vi "Tree_ItemArrayTag_Tests.vi"(11 "error in":errorcluster) -> (15 "error out":errorcluster)   [LabVIEW 2016, in "DronaTest.lvlib"]
uses:
  DronaTest.lvlib
  APIs/Stimulus/ControlValue/SetValueAuto.vi
  APIs/Stimulus/ControlValue/Controls/Tree/SetValueByItemTagArray.vi
  APIs/Assert/AssertControlValue/Equal.vi
  <vilib>/addons/_JKI Toolkits/Caraya/classes/Test/Test.lvclass
  Drona.lvlib
  <vilib>/SLL Toolkit/SLL Debug/SLL Debug.lvlib
  APIs/Assert/AssertControlValue/AssertControlValue.lvlib
  APIs/Stimulus/ControlValue/ControlValue.lvlib
  <vilib>/addons/_JKI Toolkits/Caraya/classes/Assert/Assert.lvclass
  APIs/Stimulus/ControlValue/Controls/Tree/StimulusTree.lvlib
  APIs/Get/GetControlRef/GetControlRef.lvlib
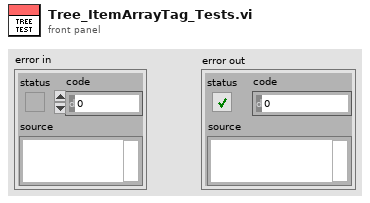
[diagram p1: front panel]
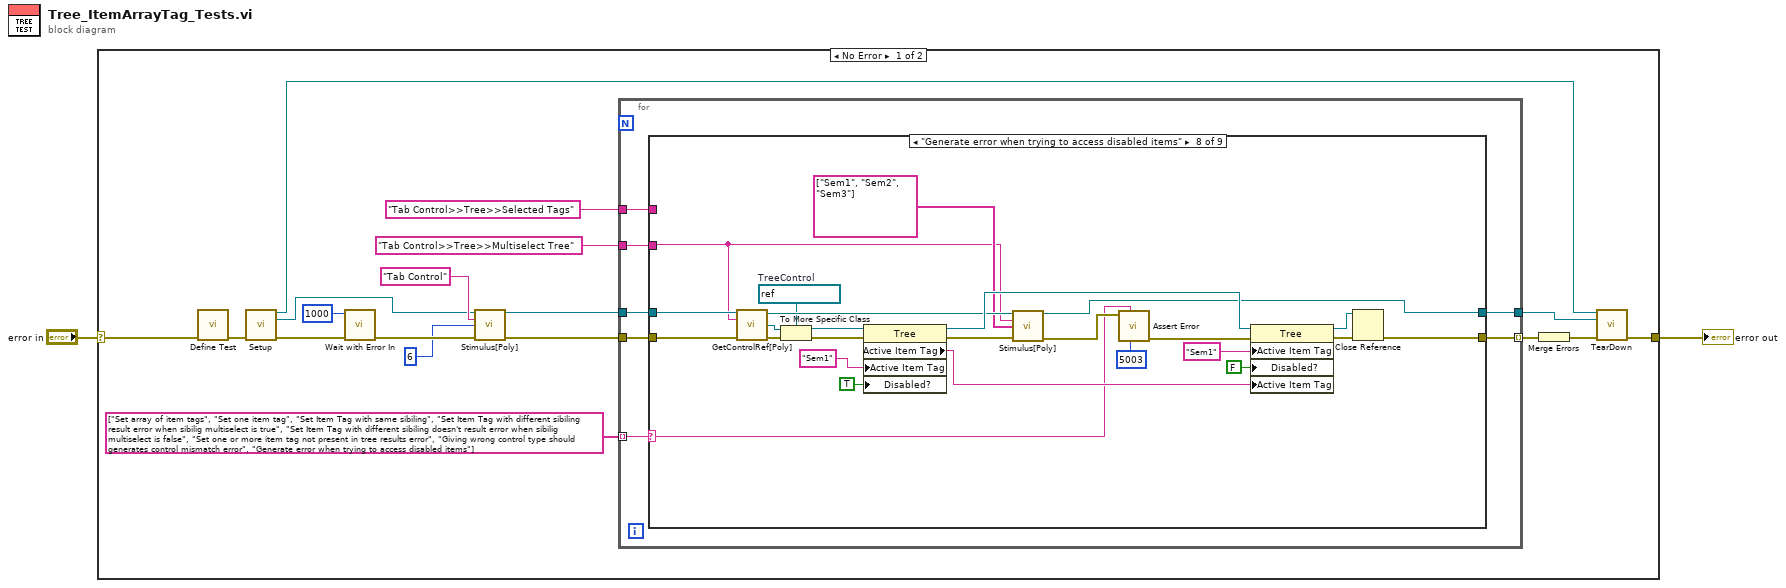
[diagram p0: block diagram]
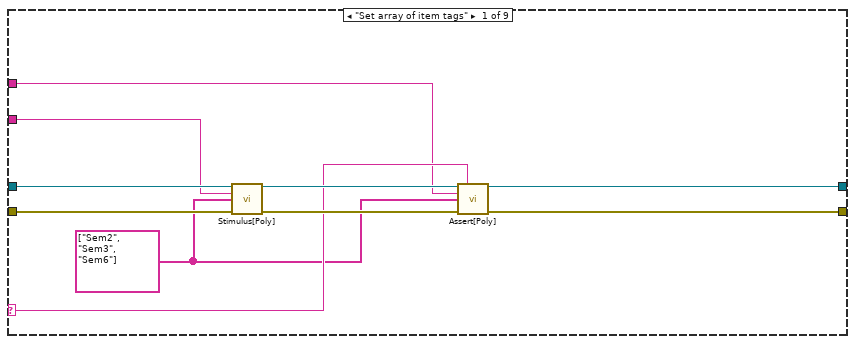
[diagram p2: hidden frame]
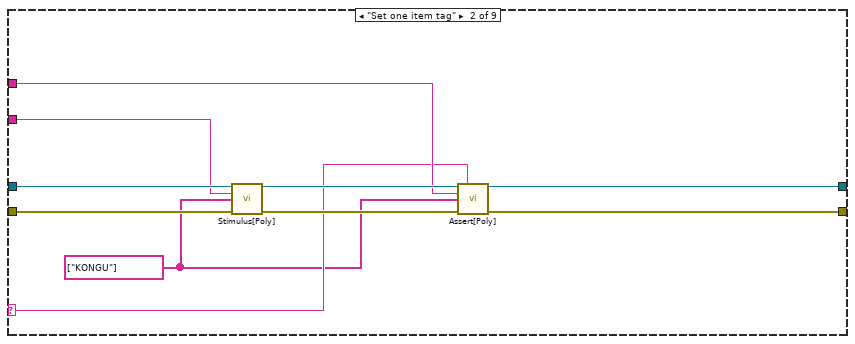
[diagram p3: hidden frame]
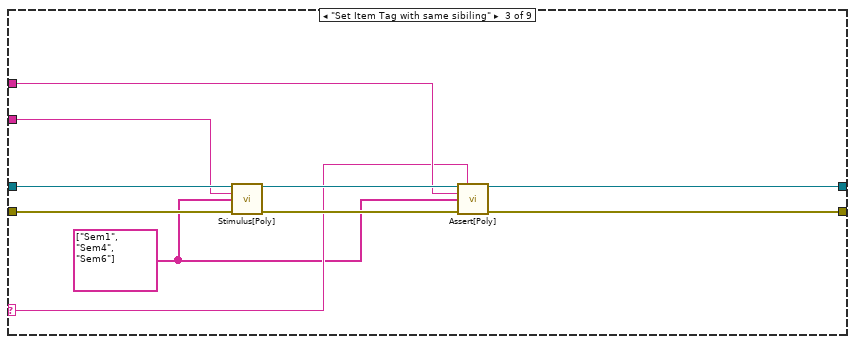
[diagram p4: hidden frame]
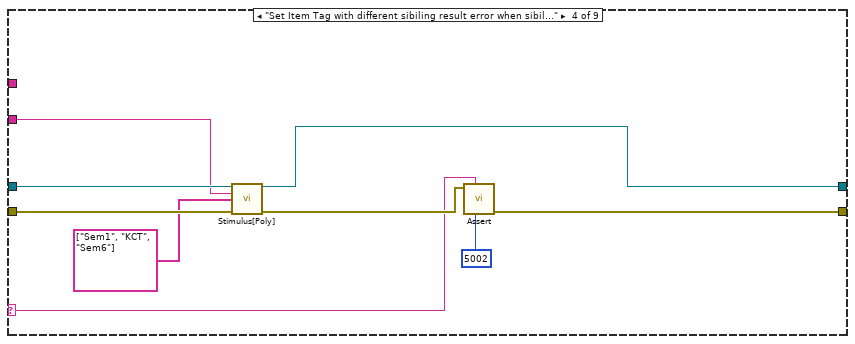
[diagram p5: hidden frame]
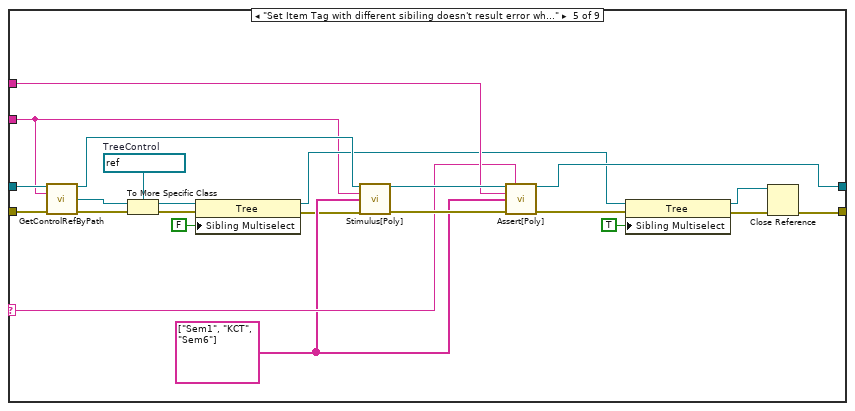
[diagram p6: hidden frame]
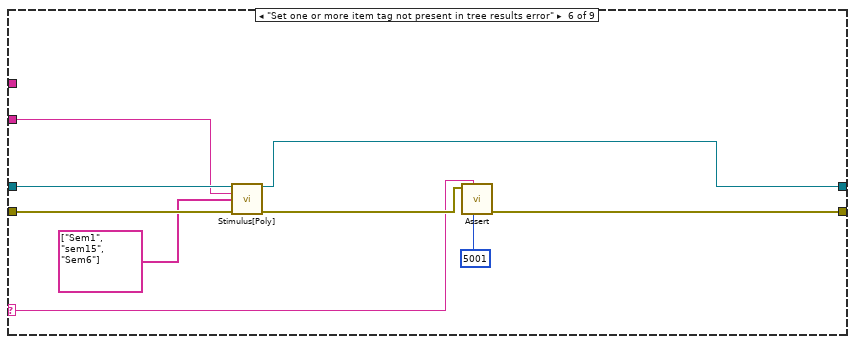
[diagram p7: hidden frame]
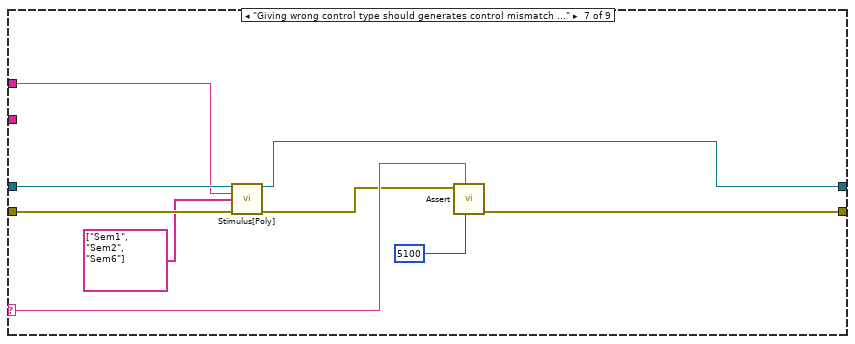
[diagram p8: hidden frame]
diagram:
  n1 = case shown="No Error" "error in" {
    selector: "error in" -> [w20 w135]
    tunnel: [w3 w135] -> w1
    frame No Error {
      n2 = call <vilib>:"Define Test.vi"("error in (no error)"=w20) -> ("error out"=w9:errorcluster)  [unwired: 9 in, 1 out]
      n3 = call "Setup.vi"("error in"=w9) -> ("Application Ref"=w4:refnum<vi>, "VI out"=w8:refnum<vi>, "error out"=w7:errorcluster)  [unwired: 12 in]
      n4 = call <vilib>:"Wait with Error In.vi"("error in (no error)"=w7, "milliseconds to wait"=u32 1000) -> ("error out"=w18:errorcluster)  [unwired: 9 in]
      n5 = call-poly "Stimulus[Poly].vi"("VI Reference In"=w8, "Control Path"="Tab Control", "Value (Signaling)"=6, "error in"=w18) -> ("VI Reference Out"=w14:refnum<vi>, "error out"=w17:errorcluster)  [unwired: 10 in]
      n6 = for {
        tunnel: w14 -> [w26]
        tunnel: "Tab Control>>Tree>>Multiselect Tree" ("Control Path") -> [w25]
        tunnel: "Tab Control>>Tree>>Selected Tags" ("Control Path") -> [w24]
        tunnel: string[] ["Set array of item tags", "Set one item tag", "Set Item Tag with same sibiling", "Set Item Tag with different sibiling result error when sibilig multiselect is true", "Set Item Tag with different sibiling doesn't result error when sibilig multiselect is false", "Set one or more item tag not present in tree results error", "Giving wrong control type should generates control mismatch error", "Generate error when trying to access disabled items"] -> [w22] mode=indexing
        tunnel: [w21] -> w5
        tunnel: w17 -> [w27]
        tunnel: [w23] -> w10 mode=indexing
        n7 = case shown="\"Generate error when trying to access disabled items\"" w22 {
          selector: w22 -> [w31 w39 w49 w61 w85 w92 w104 w110 _]
          tunnel: w27 -> [w37 w47 w57 w66 w83 w98 w107 w114 w134]
          tunnel: w26 -> [w36 w46 w56 w65 w82 w97 w106 w113 w133]
          tunnel: w25 -> [w29 w43 w53 w64 w67 w96 _ w108 _]
          tunnel: w24 -> [w30 w42 w52 _ w87 _ w100 _ _]
          tunnel: [w33 w41 w51 w59 w69 w95 w105 w112 w134] -> w23
          tunnel: [w32 w40 w50 w58 w86 w94 w103 w111 w133] -> w21
          frame "Set array of item tags" {
            w28 = string[] ["Sem2", "Sem3", "Sem6"] ("Item Name")
            n8 = call-poly "Stimulus[Poly].vi"("VI Reference In"=w36, "Control Path"=w29, "Item Tags Array"=w28, "Error In"=w37) -> ("VI Reference Out"=w34:refnum<vi>, "Error Out"=w35:errorcluster)  [unwired: 10 in]
            n9 = call-poly "Assert[Poly].vi"("VI Reference In"=w34, "Test Label"=w31, "Control Path"=w30, "Control Value"=w28, "Error In"=w35) -> ("VI Reference Out"=w32:refnum<vi>, "Error Out"=w33:errorcluster)  [unwired: 8 in, 1 out]
          }
          frame "Set one item tag" {
            w38 = string[] ["KONGU"] ("Item Name")
            n10 = call-poly "Stimulus[Poly].vi"("VI Reference In"=w46, "Control Path"=w43, "Item Tags Array"=w38, "Error In"=w47) -> ("VI Reference Out"=w44:refnum<vi>, "Error Out"=w45:errorcluster)  [unwired: 10 in]
            n11 = call-poly "Assert[Poly].vi"("VI Reference In"=w44, "Test Label"=w39, "Control Path"=w42, "Control Value"=w38, "Error In"=w45) -> ("VI Reference Out"=w40:refnum<vi>, "Error Out"=w41:errorcluster)  [unwired: 8 in, 1 out]
          }
          frame "Set Item Tag with same sibiling" {
            w48 = string[] ["Sem1", "Sem4", "Sem6"] ("Item Name")
            n12 = call-poly "Stimulus[Poly].vi"("VI Reference In"=w56, "Control Path"=w53, "Item Tags Array"=w48, "Error In"=w57) -> ("VI Reference Out"=w54:refnum<vi>, "Error Out"=w55:errorcluster)  [unwired: 10 in]
            n13 = call-poly "Assert[Poly].vi"("VI Reference In"=w54, "Test Label"=w49, "Control Path"=w52, "Control Value"=w48, "Error In"=w55) -> ("VI Reference Out"=w50:refnum<vi>, "Error Out"=w51:errorcluster)  [unwired: 8 in, 1 out]
          }
          frame "Set Item Tag with different sibiling result error when sibilig multiselect is true" {
            n14 = call-poly "Stimulus[Poly].vi"("VI Reference In"=w65, "Control Path"=w64, "Item Tags Array"=string[] ["Sem1", "KCT", "Sem6"] ("Item Name"), "Error In"=w66) -> ("VI Reference Out"=w58:refnum<vi>, "Error Out"=w62:errorcluster)  [unwired: 10 in]
            n15 = call-poly <vilib>:"Assert.vi"("error code (1)"=5002, "Label"=w61, "Error?"=w62) -> ("error out"=w59:errorcluster)  [unwired: 7 in, 1 out]
          }
          frame "Set Item Tag with different sibiling doesn't result error when sibilig multiselect is false" {
            w78 = refnum<vi> refnum  # TreeControl
            w84 = string[] ["Sem1", "KCT", "Sem6"] ("Item Name")
            n16 = call "GetControlRefByPath.vi"("VI Reference In"=w82, "Control Path"=w67, "error In"=w83) -> ("VI Reference Out"=w81:refnum<vi>, "Ctl Refnum"=w80:refnum<vi>, "error out"=w79:errorcluster)  [unwired: 10 in]
            n17 = To More Specific Class(target class=w78, reference=w80, error in=w79) -> (specific class reference=w77:refnum<vi>, error out=w76:errorcluster)
            n18 = property class="Tree"(reference=w77, error in=w76, "Sibling Multiselect"=FALSE) -> (reference out=w70:refnum<vi>, error out=w74:errorcluster)
            n19 = call-poly "Stimulus[Poly].vi"("VI Reference In"=w81, "Control Path"=w67, "Item Tags Array"=w84, "Error In"=w74) -> ("VI Reference Out"=w88:refnum<vi>, "Error Out"=w89:errorcluster)  [unwired: 10 in]
            n20 = call-poly "Assert[Poly].vi"("VI Reference In"=w88, "Test Label"=w85, "Control Path"=w87, "Control Value"=w84, "Error In"=w89) -> ("VI Reference Out"=w86:refnum<vi>, "Error Out"=w72:errorcluster)  [unwired: 8 in, 1 out]
            n21 = property class="Tree"(reference=w70, error in=w72, "Sibling Multiselect"=TRUE) -> (reference out=w68:refnum<vi>, error out=w71:errorcluster)
            n22 = Close Reference(reference=w68, error in (no error)=w71) -> (error out=w69:errorcluster)
          }
          frame "Set one or more item tag not present in tree results error" {
            n23 = call-poly "Stimulus[Poly].vi"("VI Reference In"=w97, "Control Path"=w96, "Item Tags Array"=string[] ["Sem1", "sem15", "Sem6"] ("Item Name"), "Error In"=w98) -> ("VI Reference Out"=w94:refnum<vi>, "Error Out"=w93:errorcluster)  [unwired: 10 in]
            n24 = call-poly <vilib>:"Assert.vi"("error code (1)"=5001, "Label"=w92, "Error?"=w93) -> ("error out"=w95:errorcluster)  [unwired: 7 in, 1 out]
          }
          frame "Giving wrong control type should generates control mismatch error" {
            n25 = call-poly "Stimulus[Poly].vi"("VI Reference In"=w106, "Control Path"=w100, "Item Tags Array"=string[] ["Sem1", "Sem2", "Sem6"] ("Item Name"), "Error In"=w107) -> ("VI Reference Out"=w103:refnum<vi>, "Error Out"=w102:errorcluster)  [unwired: 10 in]
            n26 = call-poly <vilib>:"Assert.vi"("error code (1)"=5100, "Label"=w104, "Error?"=w102) -> ("error out"=w105:errorcluster)  [unwired: 7 in, 1 out]
          }
          frame "Generate error when trying to access disabled items" {
            w118 = refnum<vi> refnum  # TreeControl
            n27 = call-poly "GetControlRef[Poly].vi"("VI Reference In"=w113, "Control Path"=w108, "error In"=w114) -> ("VI Reference Out"=w125:refnum<vi>, "Ctl Refnum"=w117:refnum<vi>, "error out"=w115:errorcluster)  [unwired: 10 in]
            n28 = To More Specific Class(target class=w118, reference=w117, error in=w115) -> (specific class reference=w119:refnum<vi>, error out=w116:errorcluster)
            n29 = property class="Tree"(reference=w119, error in=w116, "Active Item Tag"="Sem1" ("Active Item:Tag"), "Disabled?"=TRUE ("Active Item:Disabled?")) -> (reference out=w129:refnum<vi>, error out=w124:errorcluster, "Active Item Tag"=w130:string)
            n30 = call-poly "Stimulus[Poly].vi"("VI Reference In"=w125, "Control Path"=w108, "Item Tags Array"=string[] ["Sem1", "Sem2", "Sem3"], "Error In"=w124) -> ("VI Reference Out"=w111:refnum<vi>, "Error Out"=w126:errorcluster)  [unwired: 10 in]
            n31 = call <vilib>:"Assert Error.vi"("error code (1)"=5003, "Label"=w110, "Error?"=w126) -> ("error out"=w127:errorcluster)  [unwired: 7 in, 1 out]
            n32 = property class="Tree"(reference=w129, error in=w127, "Active Item Tag"="Sem1" ("Active Item:Tag"), "Disabled?"=FALSE ("Active Item:Disabled?"), "Active Item Tag"=w130) -> (reference out=w123:refnum<vi>, error out=w122:errorcluster)
            n33 = Close Reference(reference=w123, error in (no error)=w122) -> (error out=w112:errorcluster)
          }
          frame Default {
          }
        }
      }
      n34 = Merge Errors(w10) -> (w6:errorcluster)
      n35 = call "TearDown.vi"("Application Ref"=w4, "VI in"=w5, "error in (no error)"=w6) -> ("error out"=w3:errorcluster)  [unwired: 12 in]
    }
    frame Error {
    }
  }
  "error out" <- w1
